vi "Init Control.vi"(5 "Group":refnum<class "Group DBL.lvclass">, 6 "Period ms":i64, 7 "VolatusAPI":refnum<class "VolatusAPI.lvclass">, 8 "error in (no error)":errorcluster, 9 "Control MsgQ":refnum<class "MessageQ.lvclass">, 10 "Config Element":refnum<class "Config Element.lvclass">, 11 "Valve in":refnum<class "DiscreteRangeControl.lvclass">) -> (0 "error out":errorcluster, 3 "Valve out":refnum<class "DiscreteRangeControl.lvclass">)   [LabVIEW 2020, in "VolatusControl.lvlib" / "DiscreteRangeControl.lvclass"]
uses:
  DiscreteRangeControl.lvclass
  lv-cdm/CDM-Config/Config Element/Config Element.lvclass
  Volatus/VolatusAPI/VolatusAPI.lvclass
  Volatus/MessageQ/MessageQ.lvclass
  lv-vecto/Vecto/Group DBL/Group DBL.lvclass
  C:/dev/lv20CE/relink/lv-vecto/Vecto/Group/Group.lvclass
  DiscreteRangeControl.lvclass/DiscreteRangeControl.ctl
  lv-cdm/CDM-Config/Config Element/Owner.vi
  lv-cdm/CDM-Config/Config Manager/Lookup Descendant.vi
  lv-vecto/Vecto/Group/Group.lvclass
  lv-cdm/CDM-Config/Config Filter/Config Lookup.lvclass
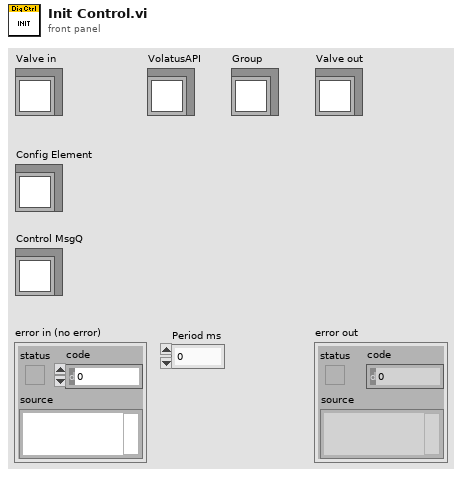
[diagram p1: front panel]
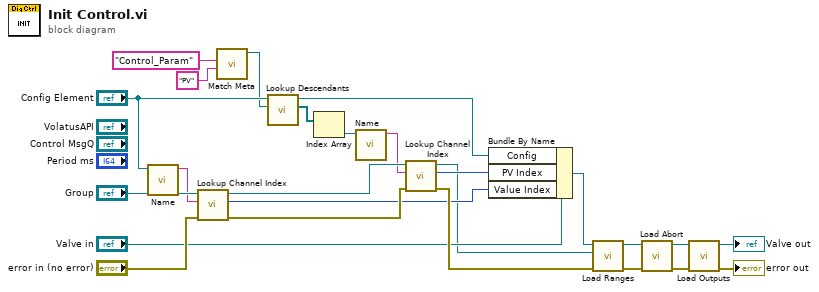
[diagram p0: block diagram]
diagram:
  n1 = call "Name.vi"("Config Element in"="Config Element") -> ("Name"=w19:string)  [unwired: 9 in, 1 out]
  n2 = call "Lookup Channel Index.vi"("error in (no error)"="error in (no error)", "Channel Name"=w19, "Group in"="Group") -> ("error out"=w24:errorcluster, "Index"=w18:i32, "Group out"=w11:refnum<class "Group DBL.lvclass">)  [unwired: 6 in]
  n3 = call "Match Meta.vi"("Value (Any)"="PV" ("Name"), "Name"="Control_Param") -> ("Config Lookup out"=w14:refnum<class "Config Lookup.lvclass">)  [unwired: 8 in, 1 out]
  n4 = call "Lookup Descendants.vi"("Lookup"=w14, "Config Element in"="Config Element") -> ("Descendants"=w13:refnum<class "Config Element.lvclass">[], "Config Element out"=w17:refnum<class "Config Element.lvclass">)  [unwired: 7 in, 1 out]
  n5 = Index Array(array=w13) -> (element=w12:refnum<class "Config Element.lvclass">)  [unwired: 1 in]
  n6 = call "Name.vi"("Config Element in"=w12) -> ("Name"=w10:string)  [unwired: 9 in, 1 out]
  n7 = call "Lookup Channel Index.vi"("error in (no error)"=w24, "Channel Name"=w10, "Group in"=w11) -> ("error out"=w25:errorcluster, "Index"=w9:i32, "Group out"=w4:refnum<class "Group DBL.lvclass">)  [unwired: 6 in]
  n8 = Bundle By Name(cluster="Valve in", "Config"=w17, "PV Index"=w9, "Value Index"=w18) -> (w3:refnum<class "DiscreteRangeControl.lvclass">)
  n9 = call "Load Ranges.vi"("error in (no error)"=w25, "Group"=w4, "DiscreteRangeControl in"=w3) -> ("error out"=w5:errorcluster, "DiscreteRangeControl out"=w6:refnum<class "DiscreteRangeControl.lvclass">)  [unwired: 7 in]
  n10 = call "Load Abort.vi"("error in (no error)"=w5, "DiscreteRangeControl in"=w6) -> ("error out"=w8:errorcluster, "DiscreteRangeControl out"=w7:refnum<class "DiscreteRangeControl.lvclass">)  [unwired: 8 in]
  n11 = call "Load Outputs.vi"("error in (no error)"=w8, "DiscreteRangeControl in"=w7) -> ("error out"=→"error out":errorcluster, "DiscreteRangeControl out"=→"Valve out":refnum<class "DiscreteRangeControl.lvclass">)  [unwired: 8 in]
